vi "Next Segment.vi"(8 "error in (no error)":errorcluster, 10 "Count":i32, 11 "MCP SSE Response in":refnum<class "MCP SSE Response.lvclass">) -> (0 "error out":errorcluster, 1 "Last?":bool, 2 "Data":string, 3 "MCP SSE Response out":refnum<class "MCP SSE Response.lvclass">)   [LabVIEW 2020, in "MCP Server.lvlib" / "MCP SSE Response.lvclass"]
doc: "Returns the next Server-Sent Event to send as one HTTP chunk. Waits on the events queue, retrying every 3 s while it times out, so the call blocks until an event exists. An empty string element, a released or invalid events queue, or an error at error in ends the stream: Last? is TRUE and Data is the SSE comment \":\" followed by a blank line. Data must not be empty there, because the IG HTTP Server writes every segment as a chunk and an empty chunk is the terminating chunk, which it writes once more afterwards. Errors from the queue itself are not passed on; error out carries error in unchanged. Count is required by the parent's interface and ignored."
uses:
  MCP SSE Response.lvclass
  MCP SSE Response.lvclass/MCP SSE Response.ctl
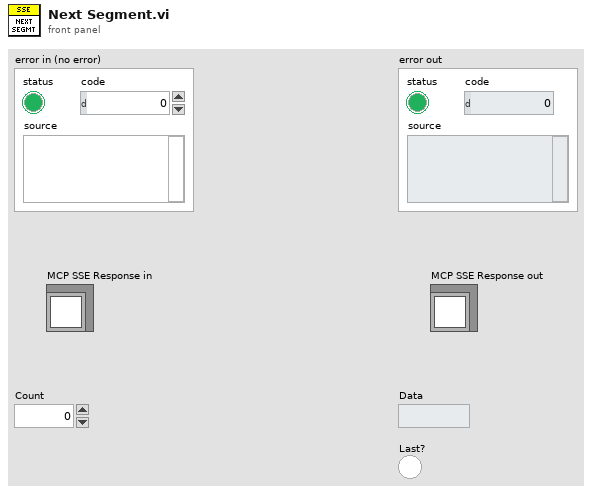
[diagram p1: front panel]
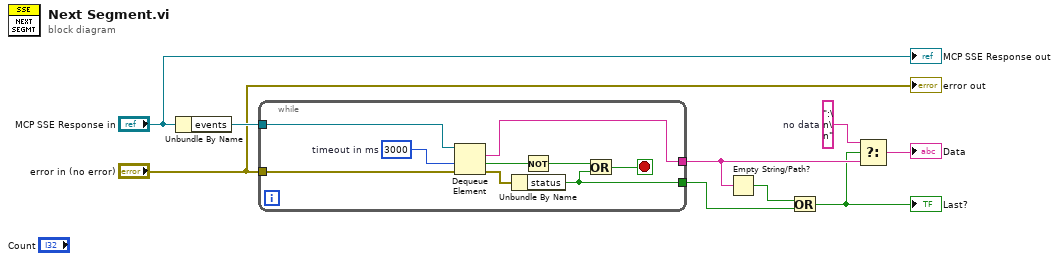
[diagram p0: block diagram]
diagram:
  w6 = ":\n\n"  # no data
  n1 = Unbundle By Name("MCP SSE Response in") -> ("events"=w9:refnum<queue>)
  n2 = while {
    tunnel: w9 -> [w18]
    tunnel: "error in (no error)" -> [w16]
    tunnel: [w11] -> w5
    tunnel: [w10] -> w7
    stop <- w12 stop-if-true
    w17 = 3000  # timeout in ms
    n3 = Dequeue Element(queue=w18, timeout in ms (-1)=w17, error in (no error)=w16) -> (element=w11:string, timed out?=w14:bool, error out=w15:errorcluster)  [unwired: 1 out]
    n4 = Unbundle By Name(w15) -> ("status"=w10:bool)
    n5 = Not(x=w14) -> (.not. x?=w13:bool)
    n6 = Or(x=w13, y=w10) -> (x .or. y?=w12:bool)
  }
  n7 = Empty String/Path?(string/path=w5) -> (empty?=w8:bool)
  n8 = Or(x=w8, y=w7) -> (x .or. y?=w1:bool)
  "Last?" <- w1
  n9 = Select(t=w6, s=w1, f=w5) -> (s? t:f=→"Data":string)
  "error out" <- "error in (no error)"
  "MCP SSE Response out" <- "MCP SSE Response in"
